vi "SCADA.vi"() -> ()   [LabVIEW 2026]
uses:
  Typedefs/BeltCtrl.ctl
  Variables/ComGlobalVars.vi
panel:
  in  "Conveyor Speed":dbl(knob) min=0.0 max=100.0 scale=0.0..100.0
  out "Classify":bool
  out "Sort":bool
  out "Idle":bool
  in  "Conveyor Control":i8(slide) min=0 max=4 step=1 scale=0.0..4.0
  in  "Stop System":bool
  out "Reject":bool
  out "Purple":bool
  out "Pink":bool
  out "Yellow":bool
  out "Throughput (Obj/min)":dbl
  out "Reject Count":i32
  out "Purple Count":i32
  out "Pink count":i32
  out "Yellow":i32
  in  "Servo Control":i16(slide)=3 caption="Slide" scale=0.0..3.0
  in  "Toggle Auto and \nManual Control":bool
  out "Live Camera Feed":T1(plugin-control)
  # "Which bin is the\nservo pointing to"
  # "What is the current state?"
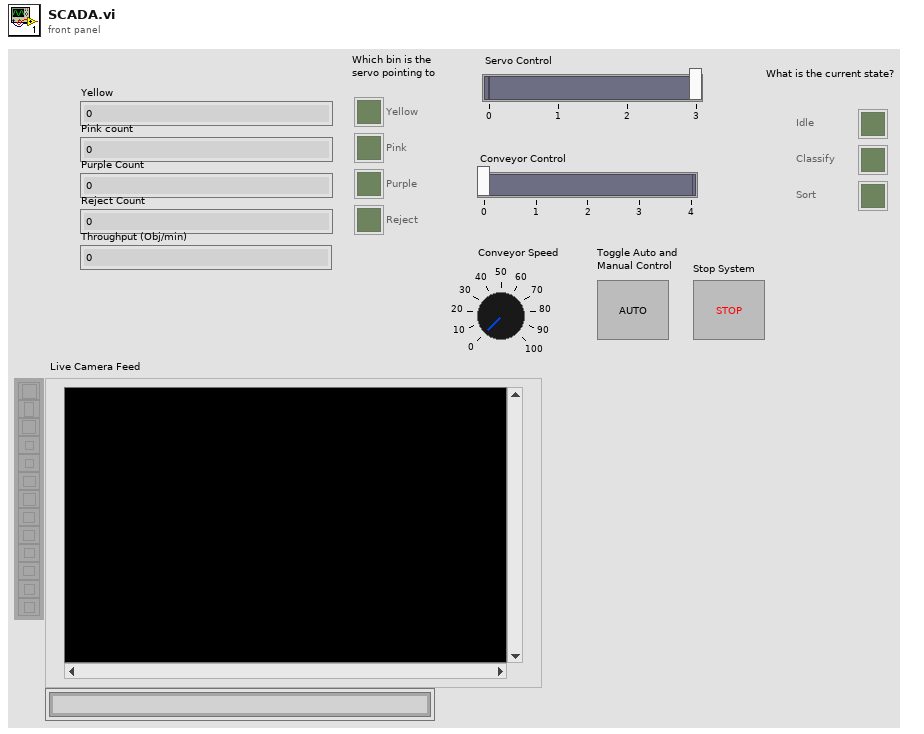
[diagram p1: front panel]
types:
  T1 = typedef "IMAQ Image.ctl" = refnum<image>
  T2 = typedef "BeltCtrl.ctl" = enum16{"Off", "Forward", "Back", "Coast", "Brake"}
  T3 = enum8{"Enabled", "Disabled", "Disabled and Grayed Out"}
  T4 = typedef "System_State.ctl" = u16
  T5 = typedef "ServoCommand.ctl" = enum16{"colour 1", "Colour2", "Colour3", "Reject"}
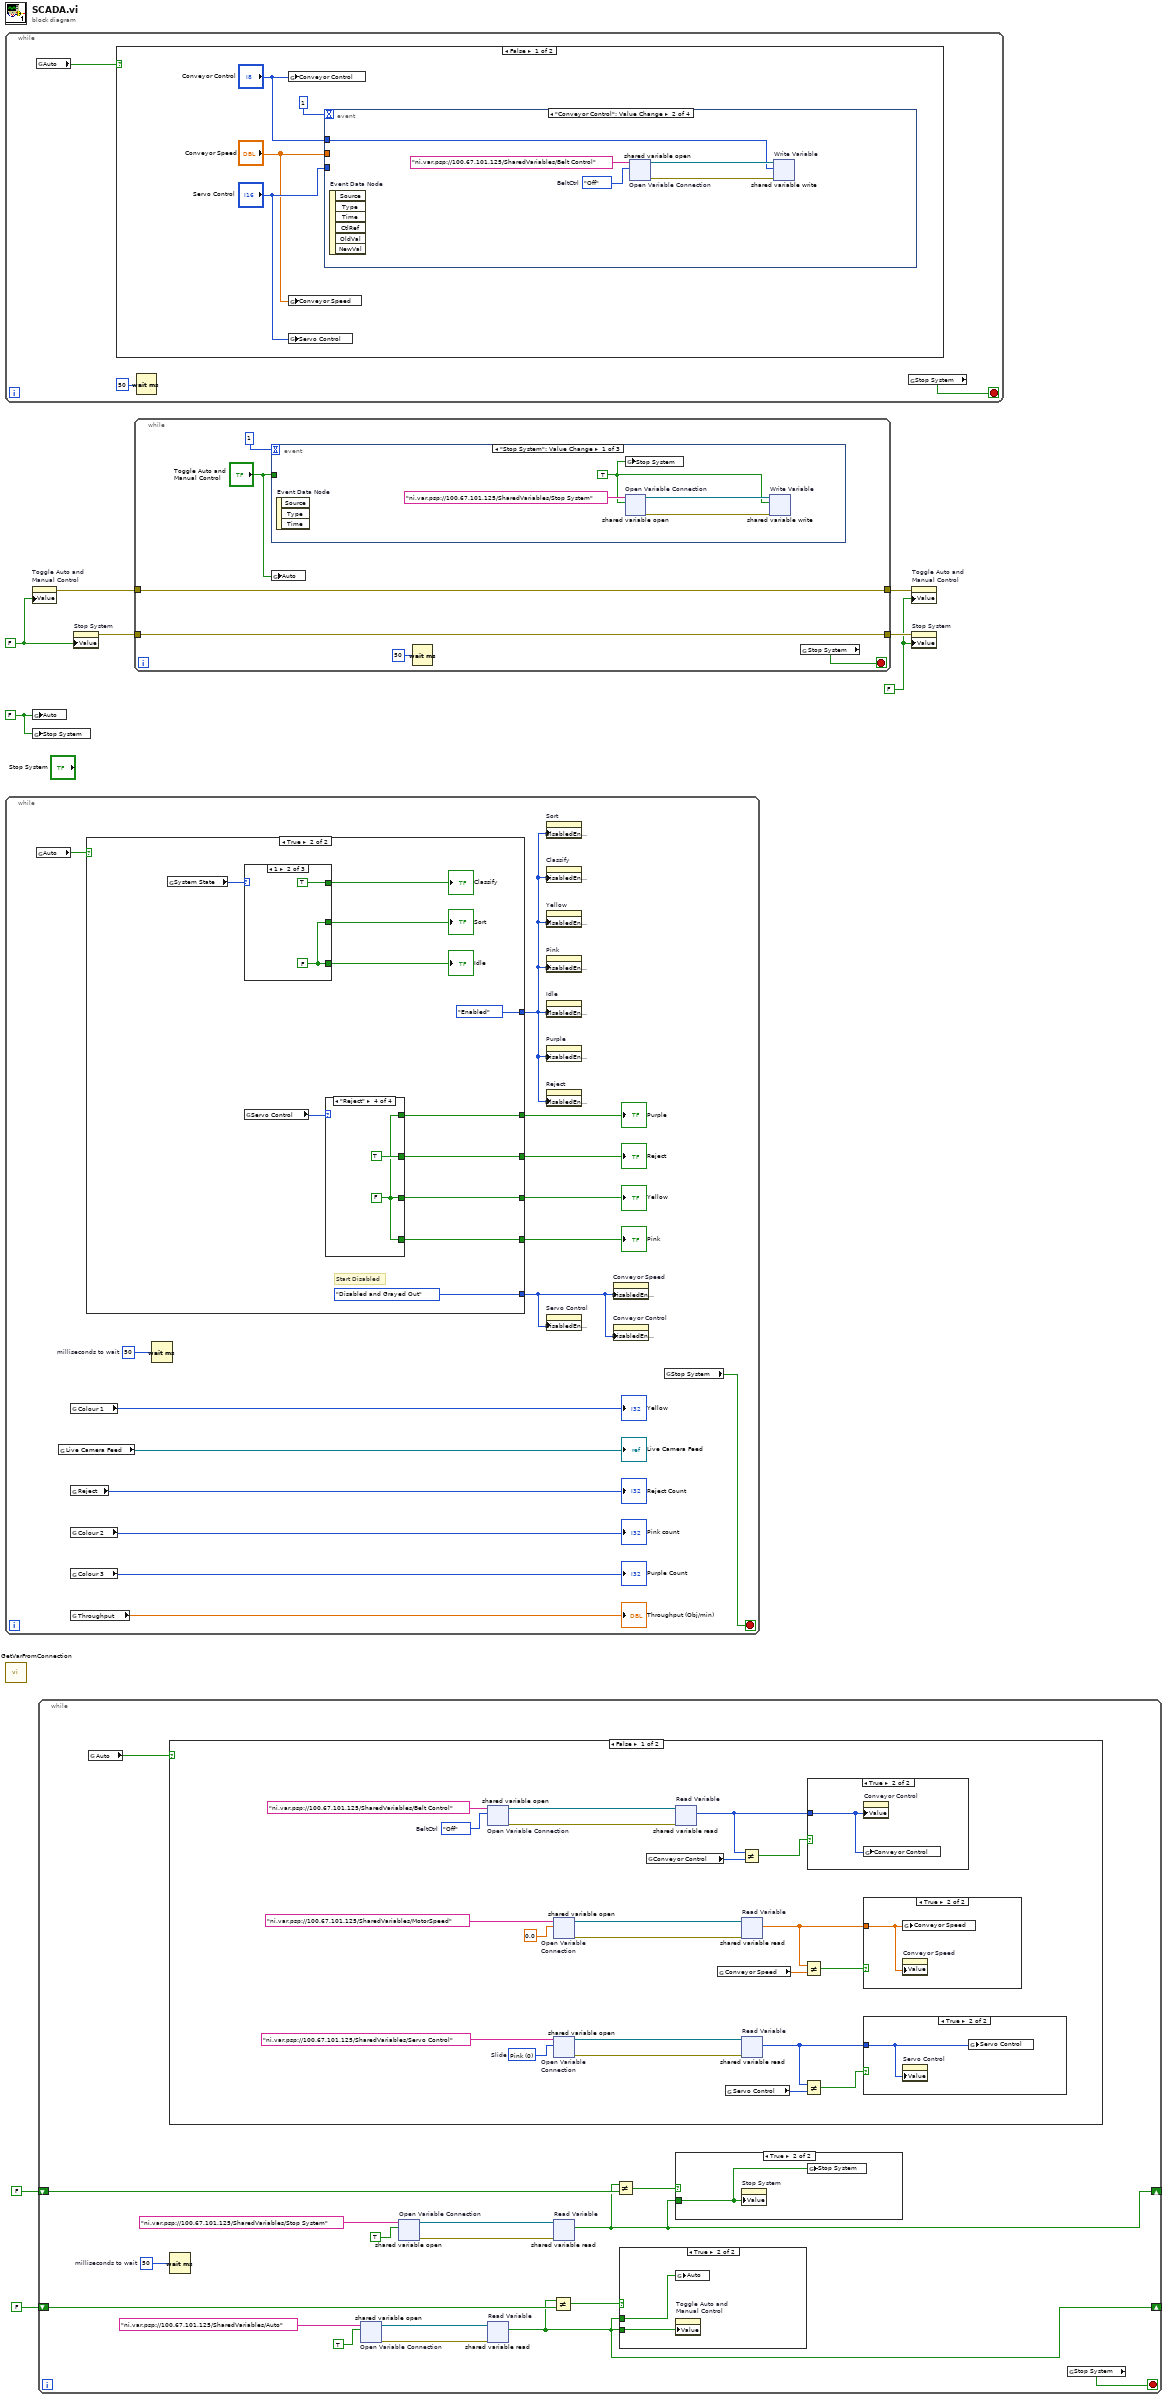
[diagram p0: block diagram]
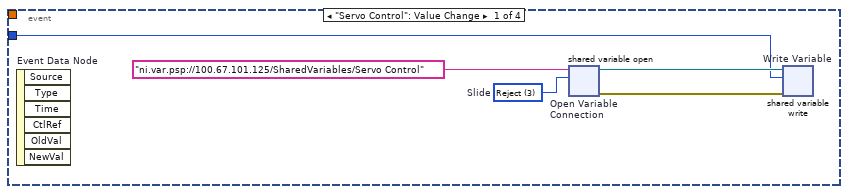
[diagram p2: hidden frame]
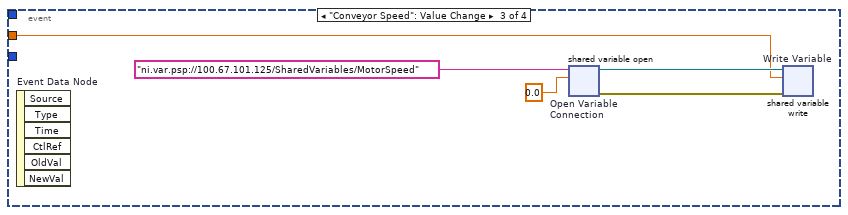
[diagram p3: hidden frame]
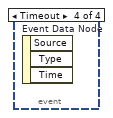
[diagram p4: hidden frame]
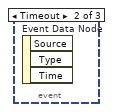
[diagram p6: hidden frame]
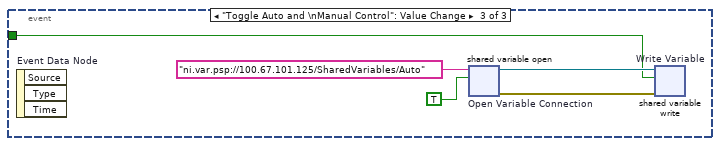
[diagram p7: hidden frame]
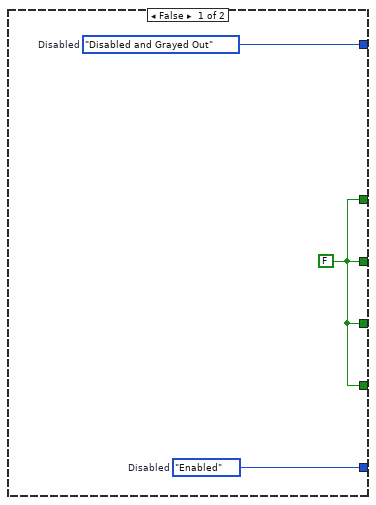
[diagram p14: hidden frame]
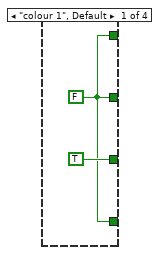
[diagram p15: hidden frame]
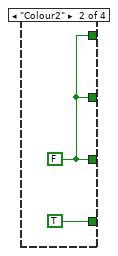
[diagram p16: hidden frame]
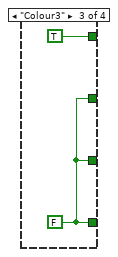
[diagram p17: hidden frame]
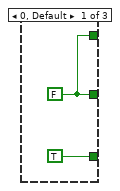
[diagram p18: hidden frame]
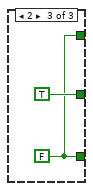
[diagram p19: hidden frame]
diagram:
  w3 = FALSE ("Stop System")
  w4 = FALSE ("Stop System")
  w7 = FALSE ("Stop System")
  n1 = while {
    stop <- w11 stop-if-true
    n2 = global read "ComGlobalVars.vi" "Auto"() -> (w12:bool)
    n3 = case shown="False" w12 {
      frame False {
        n4 = global write "ComGlobalVars.vi" "Conveyor Control"("Conveyor Control") -> ()
        n5 = global write "ComGlobalVars.vi" "Conveyor Speed"("Conveyor Speed") -> ()
        n6 = global write "ComGlobalVars.vi" "Servo Control"("Servo Control") -> ()
        n7 = event shown="[1] \"Conveyor Control\": Value Change" {
          selector: _ -> [_ _ _ _]
          dyn-events: _ -> [_ _ _ _]
          timeout: 1 -> [_ _ _ _]
          tunnel: "Conveyor Speed" -> [_ _ w27 _]
          tunnel: "Conveyor Control" -> [_ w22 _ _]
          tunnel: "Servo Control" -> [w17 _ _ _]
          event "Servo Control": Value Change {
            w18 = u16 3 items=["Pink", "Yellow", "Purple", "Reject"]  # Slide
            n8 = event-data "Event Data Node"() -> ()  [unwired: 1 in, 6 out]
            n9 = shared-variable-open "Open Variable Connection"("ni.var.psp://100.67.101.125/SharedVariables/Servo Control", w18) -> (w20:refnum<k21>, w19:errorcluster)  [unwired: 2 in]
            n10 = shared-variable-write "Write Variable"(w20, w19, w17) -> ()  [unwired: 2 out]
          }
          event "Conveyor Control": Value Change {
            w23 = BeltCtrl."Off"  # BeltCtrl
            n11 = event-data "Event Data Node"() -> ()  [unwired: 1 in, 6 out]
            n12 = shared-variable-open "Open Variable Connection"("ni.var.psp://100.67.101.125/SharedVariables/Belt Control", w23) -> (w25:refnum<k21>, w24:errorcluster)  [unwired: 2 in]
            n13 = shared-variable-write "Write Variable"(w25, w24, w22) -> ()  [unwired: 2 out]
          }
          event "Conveyor Speed": Value Change {
            n14 = event-data "Event Data Node"() -> ()  [unwired: 1 in, 6 out]
            n15 = shared-variable-open "Open Variable Connection"("ni.var.psp://100.67.101.125/SharedVariables/MotorSpeed", 0.0) -> (w29:refnum<k21>, w28:errorcluster)  [unwired: 2 in]
            n16 = shared-variable-write "Write Variable"(w29, w28, w27) -> ()  [unwired: 2 out]
          }
          event Timeout {
            n17 = event-data "Event Data Node"() -> ()  [unwired: 1 in, 3 out]
          }
        }
      }
      frame True {
      }
    }
    n18 = Wait (ms)(milliseconds to wait=u32 50) -> ()  [unwired: 1 out]
    n19 = global read "ComGlobalVars.vi" "Stop System"() -> (w11:bool)
  }
  n20 = while {
    stop <- w39 stop-if-true
    w46 = u32 50  # milliseconds to wait
    n21 = global read "ComGlobalVars.vi" "Auto"() -> (w32:bool)
    n22 = global read "ComGlobalVars.vi" "Live Camera Feed"() -> (→"Live Camera Feed":T1)
    n23 = global read "ComGlobalVars.vi" "Colour 1"() -> (→"Yellow":i32)
    n24 = global read "ComGlobalVars.vi" "Reject"() -> (→"Reject Count":i32)
    n25 = global read "ComGlobalVars.vi" "Colour 2"() -> (→"Pink count":i32)
    n26 = global read "ComGlobalVars.vi" "Colour 3"() -> (→"Purple Count":i32)
    n27 = global read "ComGlobalVars.vi" "Throughput"() -> (→"Throughput (Obj/min)":dbl)
    n28 = case shown="True" w32 {
      tunnel: [w49 w55] -> w38
      tunnel: [w49 w54] -> w37
      tunnel: [w49 w53] -> w36
      tunnel: [w49 w52] -> w35
      tunnel: [w48 T3."Enabled" ("Disabled")] -> w33
      tunnel: [w47 T3."Disabled and Grayed Out" ("Disabled")] -> w34
      frame False {
        w47 = T3."Enabled"  # Disabled
        w49 = FALSE
        w48 = T3."Disabled and Grayed Out"  # Disabled
      }
      frame True {
        # "Start Disabled"
        n29 = global read "ComGlobalVars.vi" "System State"() -> (w60:T4)
        n30 = case shown="1" w60 {
          tunnel: [TRUE w71 w73] -> w59
          tunnel: [w69 w71 TRUE] -> w58
          tunnel: [w69 TRUE w73] -> w57
          frame 0, Default {
            w69 = FALSE
          }
          frame 1 {
            w71 = FALSE
          }
          frame 2 {
            w73 = FALSE
          }
        }
        "Idle" <- w59
        "Classify" <- w57
        "Sort" <- w58
        n31 = global read "ComGlobalVars.vi" "Servo Control"() -> (w56:T5)
        n32 = case shown="\"Reject\"" w56 {
          tunnel: [TRUE w63 w65 w67] -> w55
          tunnel: [w61 TRUE w65 w67] -> w52
          tunnel: [w61 w63 TRUE w67] -> w53
          tunnel: [w61 w63 w65 TRUE] -> w54
          frame "colour 1", Default {
            w61 = FALSE
          }
          frame "Colour2" {
            w63 = FALSE
          }
          frame "Colour3" {
            w65 = FALSE
          }
          frame "Reject" {
            w67 = FALSE
          }
        }
      }
    }
    "Pink" <- w35
    "Purple" <- w36
    "Reject" <- w37
    "Yellow" <- w38
    n33 = Wait (ms)(milliseconds to wait=w46) -> ()  [unwired: 1 out]
    n34 = property on="Sort" class="Bool (strict)"("DisabledEnum"=w33) -> ()  [unwired: 2 in, 2 out]
    n35 = property on="Classify" class="Bool (strict)"("DisabledEnum"=w33) -> ()  [unwired: 2 in, 2 out]
    n36 = property on="Yellow" class="Bool (strict)"("DisabledEnum"=w33) -> ()  [unwired: 2 in, 2 out]
    n37 = property on="Pink" class="Bool (strict)"("DisabledEnum"=w33) -> ()  [unwired: 2 in, 2 out]
    n38 = property on="Idle" class="Bool (strict)"("DisabledEnum"=w33) -> ()  [unwired: 2 in, 2 out]
    n39 = property on="Purple" class="Bool (strict)"("DisabledEnum"=w33) -> ()  [unwired: 2 in, 2 out]
    n40 = property on="Reject" class="Bool (strict)"("DisabledEnum"=w33) -> ()  [unwired: 2 in, 2 out]
    n41 = property on="Servo Control" class="Slide (strict)"("DisabledEnum"=w34) -> ()  [unwired: 2 in, 2 out]
    n42 = property on="Conveyor Speed" class="Knob (strict)"("DisabledEnum"=w34) -> ()  [unwired: 2 in, 2 out]
    n43 = property on="Conveyor Control" class="Slide (strict)"("DisabledEnum"=w34) -> ()  [unwired: 2 in, 2 out]
    n44 = global read "ComGlobalVars.vi" "Stop System"() -> (w39:bool)
  }
  n45 = call "GetVarFromConnection.vi"() -> ()  [unwired: 12 in]
  n46 = property on="Toggle Auto and \nManual Control" class="Bool (strict)"("Value"=w7) -> (error out=w6:errorcluster)  [unwired: 2 in, 1 out]
  n47 = global write "ComGlobalVars.vi" "Auto"(w3) -> ()
  n48 = global write "ComGlobalVars.vi" "Stop System"(w3) -> ()
  n49 = while {
    shift-right: [w77] -> _
    shift-left: FALSE -> [w78]
    shift-right: [w75] -> _
    shift-left: FALSE -> [w76]
    stop <- w80 stop-if-true
    w86 = u32 50  # milliseconds to wait
    n50 = global read "ComGlobalVars.vi" "Auto"() -> (w79:bool)
    n51 = case shown="False" w79 {
      frame False {
        w92 = BeltCtrl."Off"  # BeltCtrl
        w106 = u16 0 items=["Pink", "Yellow", "Purple", "Reject"]  # Slide
        n52 = shared-variable-open "Open Variable Connection"("ni.var.psp://100.67.101.125/SharedVariables/Belt Control", w92) -> (w96:refnum<k21>, w97:errorcluster)  [unwired: 2 in]
        n53 = shared-variable-open "Open Variable Connection"("ni.var.psp://100.67.101.125/SharedVariables/MotorSpeed", 0.0) -> (w101:refnum<k21>, w102:errorcluster)  [unwired: 2 in]
        n54 = shared-variable-open "Open Variable Connection"("ni.var.psp://100.67.101.125/SharedVariables/Servo Control", w106) -> (w108:refnum<k21>, w109:errorcluster)  [unwired: 2 in]
        n55 = global read "ComGlobalVars.vi" "Conveyor Control"() -> (w100:T2)
        n56 = shared-variable-read "Read Variable"(w96, w97) -> (w99:T2)  [unwired: 3 out]
        n57 = global read "ComGlobalVars.vi" "Conveyor Speed"() -> (w104:dbl)
        n58 = global read "ComGlobalVars.vi" "Servo Control"() -> (w110:T5)
        n59 = Not Equal?(x=w99, y=w100) -> (x != y?=w98:bool)
        n60 = shared-variable-read "Read Variable"(w101, w102) -> (w103:dbl)  [unwired: 3 out]
        n61 = shared-variable-read "Read Variable"(w108, w109) -> (w112:u16)  [unwired: 3 out]
        n62 = Not Equal?(x=w103, y=w104) -> (x != y?=w105:bool)
        n63 = Not Equal?(x=w112, y=w110) -> (x != y?=w111:bool)
        n64 = case shown="True" w98 {
          tunnel: w99 -> [_ w114]
          frame False {
          }
          frame True {
            n65 = property on="Conveyor Control" class="Slide (strict)"("Value"=w114) -> ()  [unwired: 2 in, 2 out]
            n66 = global write "ComGlobalVars.vi" "Conveyor Control"(w114) -> ()
          }
        }
        n67 = case shown="True" w105 {
          tunnel: w103 -> [_ w113]
          frame False {
          }
          frame True {
            n68 = global write "ComGlobalVars.vi" "Conveyor Speed"(w113) -> ()
            n69 = property on="Conveyor Speed" class="Knob (strict)"("Value"=w113) -> ()  [unwired: 2 in, 2 out]
          }
        }
        n70 = case shown="True" w111 {
          tunnel: w112 -> [_ w115]
          frame False {
          }
          frame True {
            n71 = property on="Servo Control" class="Slide (strict)"("Value"=w115) -> ()  [unwired: 2 in, 2 out]
            n72 = global write "ComGlobalVars.vi" "Servo Control"(w115) -> ()
          }
        }
      }
      frame True {
      }
    }
    n73 = Wait (ms)(milliseconds to wait=w86) -> ()  [unwired: 1 out]
    n74 = shared-variable-open "Open Variable Connection"("ni.var.psp://100.67.101.125/SharedVariables/Auto", TRUE) -> (w89:refnum<k21>, w88:errorcluster)  [unwired: 2 in]
    n75 = shared-variable-open "Open Variable Connection"("ni.var.psp://100.67.101.125/SharedVariables/Stop System", TRUE) -> (w84:refnum<k21>, w85:errorcluster)  [unwired: 2 in]
    n76 = shared-variable-read "Read Variable"(w89, w88) -> (w75:bool)  [unwired: 3 out]
    n77 = Not Equal?(x=w75, y=w76) -> (x != y?=w87:bool)
    n78 = shared-variable-read "Read Variable"(w84, w85) -> (w77:bool)  [unwired: 3 out]
    n79 = Not Equal?(x=w77, y=w78) -> (x != y?=w81:bool)
    n80 = case shown="True" w87 {
      tunnel: w75 -> [_ w118]
      tunnel: w75 -> [_ w117]
      frame False {
      }
      frame True {
        n81 = global write "ComGlobalVars.vi" "Auto"(w118) -> ()
        n82 = property on="Toggle Auto and \nManual Control" class="Bool (strict)"("Value"=w117) -> ()  [unwired: 2 in, 2 out]
      }
    }
    n83 = case shown="True" w81 {
      tunnel: w77 -> [_ w116]
      frame False {
      }
      frame True {
        n84 = property on="Stop System" class="Bool (strict)"("Value"=w116) -> ()  [unwired: 2 in, 2 out]
        n85 = global write "ComGlobalVars.vi" "Stop System"(w116) -> ()
      }
    }
    n86 = global read "ComGlobalVars.vi" "Stop System"() -> (w80:bool)
  }
  n87 = property on="Stop System" class="Bool (strict)"("Value"=w7) -> (error out=w9:errorcluster)  [unwired: 2 in, 1 out]
  n88 = while {
    tunnel: w9 -> [w121]
    tunnel: [w121] -> w8
    tunnel: w6 -> [w120]
    tunnel: [w120] -> w5
    stop <- w123 stop-if-true
    n89 = event shown="[0] \"Stop System\": Value Change" {
      selector: _ -> [_ _ _]
      dyn-events: _ -> [_ _ _]
      timeout: 1 -> [_ _ _]
      tunnel: "Toggle Auto and \nManual Control" -> [_ _ w129]
      event "Stop System": Value Change {
        w125 = TRUE
        n90 = event-data "Event Data Node"() -> ()  [unwired: 1 in, 3 out]
        n91 = global write "ComGlobalVars.vi" "Stop System"(w125) -> ()
        n92 = shared-variable-open "Open Variable Connection"("ni.var.psp://100.67.101.125/SharedVariables/Stop System", w125) -> (w128:refnum<k21>, w127:errorcluster)  [unwired: 2 in]
        n93 = shared-variable-write "Write Variable"(w128, w127, w125) -> ()  [unwired: 2 out]
      }
      event Timeout {
        n94 = event-data "Event Data Node"() -> ()  [unwired: 1 in, 3 out]
      }
      event "Toggle Auto and \nManual Control": Value Change {
        n95 = event-data "Event Data Node"() -> ()  [unwired: 1 in, 3 out]
        n96 = shared-variable-open "Open Variable Connection"("ni.var.psp://100.67.101.125/SharedVariables/Auto", TRUE) -> (w132:refnum<k21>, w133:errorcluster)  [unwired: 2 in]
        n97 = shared-variable-write "Write Variable"(w132, w133, w129) -> ()  [unwired: 2 out]
      }
    }
    n98 = global write "ComGlobalVars.vi" "Auto"("Toggle Auto and \nManual Control") -> ()
    n99 = Wait (ms)(milliseconds to wait=u32 50) -> ()  [unwired: 1 out]
    n100 = global read "ComGlobalVars.vi" "Stop System"() -> (w123:bool)
  }
  n101 = property on="Toggle Auto and \nManual Control" class="Bool (strict)"(error in=w5, "Value"=w4) -> ()  [unwired: 1 in, 2 out]
  n102 = property on="Stop System" class="Bool (strict)"(error in=w8, "Value"=w4) -> ()  [unwired: 1 in, 2 out]
